vi "Remove_empty_all.vi"(11 "ARR_in":string[][](array[string])) -> (3 "ARR_out":string[][](array[string]))   [LabVIEW 2025, in "Procotol_class.lvclass"]
uses:
  Procotol_class.lvclass
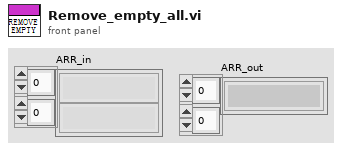
[diagram p1: front panel]
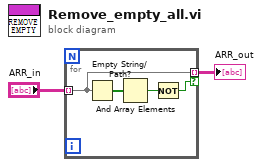
[diagram p0: block diagram]
diagram:
  n1 = for {
    tunnel: "ARR_in" -> [w5] mode=indexing
    tunnel: [w5] -> w1 mode=indexing if=w3
    n2 = Empty String/Path?(string/path=w5) -> (empty?=w6:bool[])
    n3 = And Array Elements(Boolean array=w6) -> (logical AND=w4:bool)
    n4 = Not(x=w4) -> (.not. x?=w3:bool)
  }
  "ARR_out" <- w1
